vi "Create Enum Mapper.vi"(8 "error in":errorcluster, 9 "format string":string, 10 "RPC Message Name":string, 11 "Library item in":refnum<vi>) -> (0 "error out":errorcluster, 2 "VI out":refnum<vi>, 3 "Library item out":refnum<vi>)   [LabVIEW 2019, in "gRPC Template Creation Utility.lvlib"]
uses:
  gRPC Template Creation Utility.lvlib
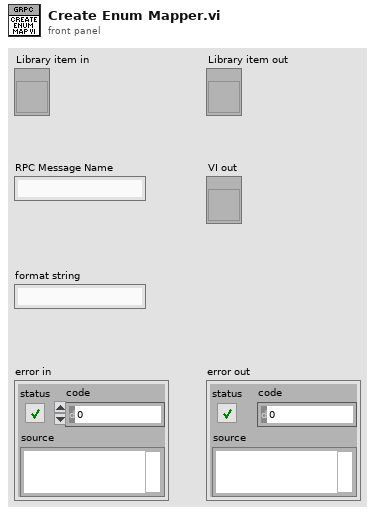
[diagram p1: front panel]
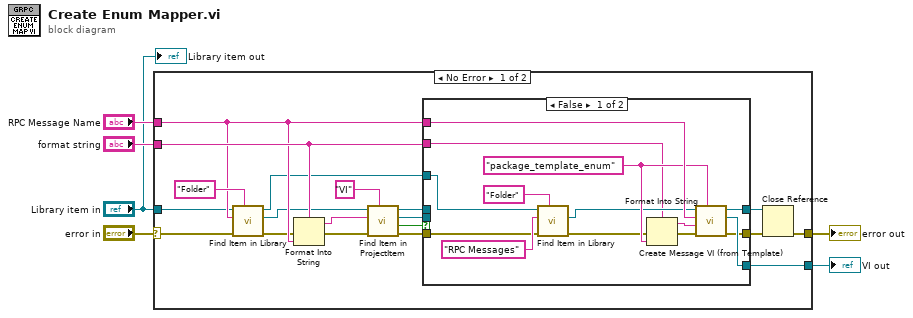
[diagram p0: block diagram]
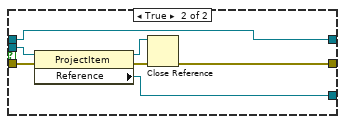
[diagram p2: hidden frame]
diagram:
  n1 = case shown="No Error" "error in" {
    selector: "error in" -> [w13 w47]
    tunnel: [w25 _] -> w6
    tunnel: [w7 w47] -> w5
    tunnel: "RPC Message Name" -> [w15 _]
    tunnel: "format string" -> [w18 _]
    tunnel: "Library item in" -> [w14 _]
    frame No Error {
      n2 = call "Find Item in Library.vi"("Item Type"="Folder", "error in (no error)"=w13, "Item Name"=w15, "Library item in"=w14) -> ("error out"=w12:errorcluster, "Project Item (Library Item)"=w10:refnum<vi>, "Library item out"=w11:refnum<vi>)  [unwired: 4 in, 1 out]
      n3 = Format Into String(format string=w18, error in=w12, w15) -> (resulting string=w19:string, error out=w17:errorcluster)  [unwired: 1 in]
      n4 = call "Find Item in ProjectItem.vi"("Item Type"="VI", "error in (no error)"=w17, "Name"=w19, "ProjectItem in"=w10) -> ("error out"=w21:errorcluster, "Found ?"=w22:bool, "Item Refnum out"=w20:refnum<vi>, "ProjectItem out"=w23:refnum<vi>)  [unwired: 4 in]
      n5 = case shown="False" w22 {
        tunnel: [w37 w45] -> w25
        tunnel: [w38 w44] -> w9
        tunnel: w21 -> [w28 w41]
        tunnel: [w36 w40] -> w8
        tunnel: w23 -> [_ w44]
        tunnel: w20 -> [_ w46]
        tunnel: w15 -> [w39 _]
        tunnel: w18 -> [w26 _]
        tunnel: w11 -> [w29 _]
        frame False {
          w35 = "package_template_enum" ("replace string in template")
          n6 = call "Find Item in Library.vi"("Item Type"="Folder", "error in (no error)"=w28, "Item Name"="RPC Messages", "Library item in"=w29) -> ("error out"=w27:errorcluster, "Project Item (Library Item)"=w30:refnum<vi>)  [unwired: 4 in, 2 out]
          n7 = Format Into String(format string=w26, error in=w27, w35) -> (resulting string=w34:string, error out=w33:errorcluster)  [unwired: 1 in]
          n8 = call "Create Message VI (from Template).vi"("replace string in template"=w35, "error in (no error)"=w33, "template VI name"=w34, "RPC Message Name"=w39, "RPC Messages Folder (ProjectItem) in"=w30) -> ("error out"=w36:errorcluster, "Getter VI out"=w37:refnum<vi>, "RPC Messages Folder (ProjectItem) out"=w38:refnum<vi>)  [unwired: 3 in, 1 out]
        }
        frame True {
          n9 = property class="ProjectItem"(reference=w46, error in=w41) -> (reference out=w42:refnum<vi>, error out=w43:errorcluster, "Reference"=w45:refnum<vi>)
          n10 = Close Reference(reference=w42, error in (no error)=w43) -> (error out=w40:errorcluster)
        }
      }
      n11 = Close Reference(reference=w9, error in (no error)=w8) -> (error out=w7:errorcluster)
    }
    frame Error {
    }
  }
  "error out" <- w5
  "VI out" <- w6
  "Library item out" <- "Library item in"
